vi "IOBlockWithMenu.vi"(0 "IP":string, 1 "Main GUI Path":string, 2 "Ctl Refnum":refnum<vi>) -> ()   [LabVIEW 2024]
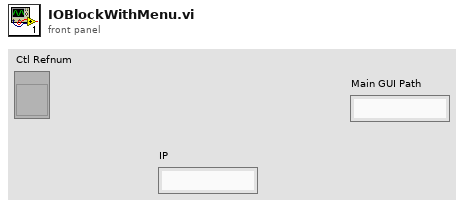
[diagram p1: front panel]
types:
  T1 = enum32{"Invalid", "Standard", "Closed", "Hidden", "Minimized", "Maximized"}
  T2 = typedef "LVPoint32TypeDef.ctl" = cluster{"Horizontal":i32, "Vertical":i32}
  T3 = typedef "LVRectTypeDef.ctl" = cluster{"Left":i16, "Top":i16, "Right":i16, "Bottom":i16}
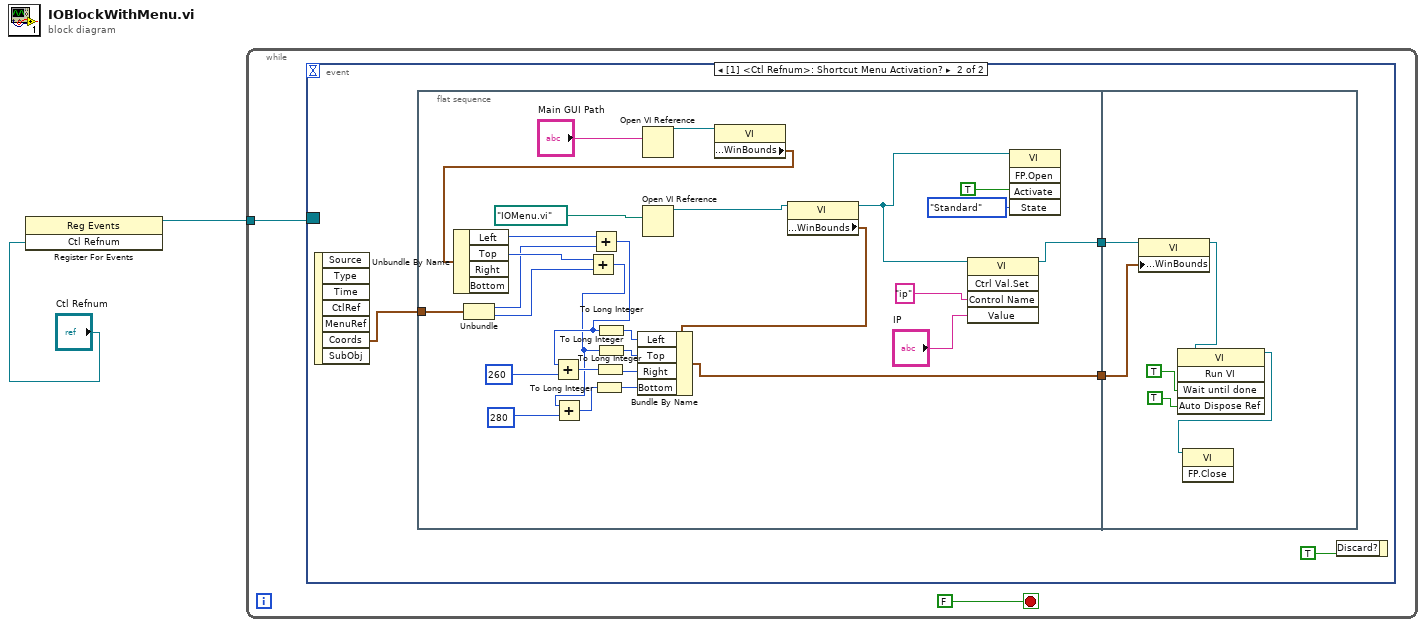
[diagram p0: block diagram]
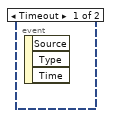
[diagram p2: hidden frame]
diagram:
  n1 = register-events("Ctl Refnum") -> (reference out=w1:refnum<event-registration>)  [unwired: 2 in, 1 out]
  n2 = while {
    tunnel: w1 -> [w3]
    stop <- FALSE stop-if-true
    n3 = event shown="[1] <Ctl Refnum>: Shortcut Menu Activation?" {
      selector: w3 -> [_ _]
      dyn-events: _ -> [_ _]
      timeout: _ -> [_ _]
      event Timeout {
        n4 = event-data() -> ()  [unwired: 1 in, 3 out]
      }
      event Shortcut Menu Activation? {
        n5 = event-data() -> ("Coords"=w6:T2)  [unwired: 1 in, 6 out]
        n6 = flat-sequence {
          tunnel: [w13] -> w8
          tunnel: [w18] -> w7
          tunnel: w6 -> [w11]
          tunnel: w8 -> [w42]
          tunnel: w7 -> [w41]
          frame #0 {
            n7 = Unbundle(w11) -> ("Horizontal"=w29:i32, "Vertical"=w31:i32)
            n8 = Open VI Reference(vi path="Main GUI Path") -> (vi reference=w24:refnum<vi>)  [unwired: 5 in, 1 out]
            n9 = Open VI Reference(vi path=path "IOMenu.vi") -> (vi reference=w17:refnum<vi>)  [unwired: 5 in, 1 out]
            n10 = property class="VI"(reference=w24) -> ("Front Panel.WinBounds"=w25:T3)  [unwired: 1 in, 2 out]
            n11 = Unbundle By Name(w25) -> ("Left"=w28:i16, "Top"=w30:i16)  [unwired: 2 out]
            n12 = Add(x=w30, y=w31) -> (x+y=w21:i32)
            n13 = Add(x=w21, y=280) -> (x+y=w19:i32)
            n14 = Add(x=w28, y=w29) -> (x+y=w23:i32)
            n15 = Add(x=w23, y=260) -> (x+y=w26:i32)
            n16 = To Long Integer(number=w19) -> (32bit integer=w32:i32)
            n17 = To Long Integer(number=w26) -> (32bit integer=w33:i32)
            n18 = To Long Integer(number=w23) -> (32bit integer=w35:i32)
            n19 = To Long Integer(number=w21) -> (32bit integer=w34:i32)
            n20 = property class="VI"(reference=w17) -> (reference out=w14:refnum<vi>, "Front Panel.WinBounds"=w27:T3)  [unwired: 1 in, 1 out]
            n21 = Bundle By Name(cluster=w27, "Left"=w35, "Top"=w34, "Right"=w33, "Bottom"=w32) -> (w18:T3)
            n22 = invoke class="VI" method="Ctrl Val.Set"(reference=w14, "Control Name"="ip", "Value"="IP") -> (reference out=w13:refnum<vi>)  [unwired: 2 in, 4 out]
            n23 = invoke class="VI" method="FP.Open"(reference=w14, "Activate"=TRUE ("Activate?"), "State"=T1."Standard") -> ()  [unwired: 2 in, 5 out]
          }
          frame #1 {
            n24 = property class="VI"(reference=w42, "Front Panel.WinBounds"=w41) -> (reference out=w38:refnum<vi>)  [unwired: 1 in, 1 out]
            n25 = invoke class="VI" method="Run VI"(reference=w38, "Wait until done"=TRUE ("Wait Until Done"), "Auto Dispose Ref"=TRUE ("Auto Dispose Reference")) -> (reference out=w37:refnum<vi>)  [unwired: 2 in, 4 out]
            n26 = invoke class="VI" method="FP.Close"(reference=w37) -> ()  [unwired: 2 in, 3 out]
          }
        }
        n27 = event-data("Discard?"=TRUE) -> ()  [unwired: 1 in, 1 out]
      }
    }
  }
